vi "Load ProtoFile.vi"(0 "protoFile ref in":u64, 1 "File Base path":path, 2 "File Name":string, 3 "error in (no error)":errorcluster) -> (7 "protoFile ref out":u64, 10 "error out":errorcluster)   [LabVIEW 2019, in "gRPC Template Creation Utility.lvlib"]
uses:
  gRPC Template Creation Utility.lvlib
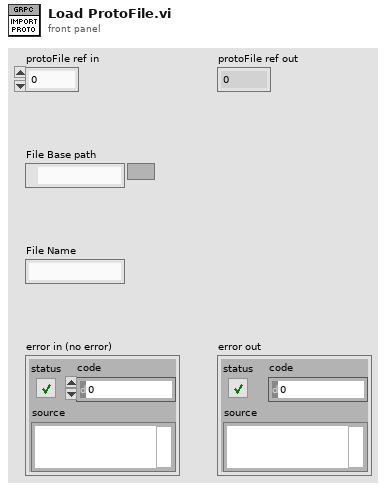
[diagram p1: front panel]
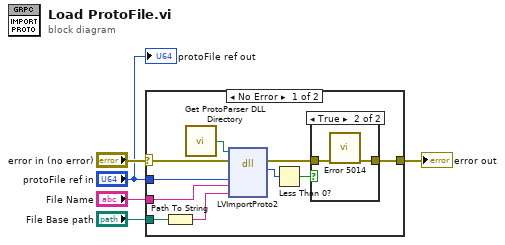
[diagram p0: block diagram]
diagram:
  n1 = case shown="No Error" "error in (no error)" {
    selector: "error in (no error)" -> [w14 w19]
    tunnel: "File Name" -> [w15 _]
    tunnel: [w11 w19] -> w3
    tunnel: "protoFile ref in" -> [w8 _]
    tunnel: "File Base path" -> [w7 _]
    frame No Error {
      n2 = Path To String(path=w7) -> (string=w6:string)
      n3 = call "Get ProtoParser DLL Directory.vi"() -> ("Proto Parser Directory"=w13:path)
      n4 = dll-call lib="?" fn="LVImportProto2"(path in=w13, error in=w14, "protoRef"=w8, "protoName"=w15, "SearchPaths"=w6) -> (error out=w12:errorcluster, "return type"=w10:i32)  [unwired: 4 in, 1 out]
      n5 = Less Than 0?(x=w10) -> (x < 0?=w9:bool)
      n6 = case shown="True" w9 {
        tunnel: w12 -> [w16 w18]
        tunnel: [w16 w17] -> w11
        frame False {
        }
        frame True {
          n7 = call "Error 5014.vi"("error in (no error)"=w18) -> ("error out"=w17:errorcluster)  [unwired: 10 in]
        }
      }
    }
    frame Error {
    }
  }
  "error out" <- w3
  "protoFile ref out" <- "protoFile ref in"
